vi "Add Parameter.vi"(8 "error in":errorcluster, 9 "parameter encoding":T1={"start index"=0, "size"=8, "encoding"=enum."BCD", "signed"=FALSE, "scale multiplier"=1.0, "scale offset"=0.0}, 10 "parameter definition":T4, 11 "label in":T3 format="%.0x") -> (0 "error out":errorcluster, 2 "parameter":T3 format="%.0x", 3 "label out":T3 format="%.0x")   [LabVIEW 2023, in "Ballard ARINC 429 Scripting.lvlib"]
doc: "Adds the specified <b>parameter definition</b> with <b>parameter encoding</b> to the system definition in the 'Word' subsection of <b>label in</b>. Returns the newly added <b>parameter</b> reference."
uses:
  Ballard ARINC 429 Scripting.lvlib
  <vilib>/NI VeriStand/Custom Device API/Custom Device Item Ref.ctl
  Shared/Parameter Definition.ctl
  <vilib>/NI/NI VeriStand Encoding and Decoding/Encoding.ctl
  <vilib>/NI VeriStand/Custom Device API/Custom Device Channel.ctl
  <vilib>/NI VeriStand/Custom Device API/Custom Device Channel Type.ctl
  Constants.vi
  <vilib>/NI VeriStand/Custom Device API/Custom Device API.lvlib
  ARINC 429/ARINC 429 Scripting.lvlib
  <vilib>/NI VeriStand/Custom Device Offline API/Custom Device Offline API.lvlib
  <vilib>/NI/NI VeriStand Encoding and Decoding/Encoding and Decoding.lvlib
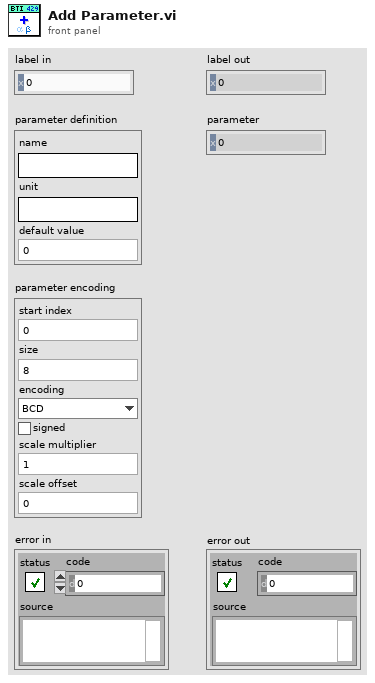
[diagram p1: front panel]
types:
  T1 = typedef "Parameter Definition.ctl" = cluster{"start index":i32, "size":i32, "encoding":T2, "signed":bool, "scale multiplier":dbl, "scale offset":dbl}
  T2 = typedef "Encoding and Decoding.lvlib/Encoding.ctl" = enum16{"BNR", "BCD", "Discrete"}
  T3 = typedef "Custom Device API.lvlib/Custom Device Item Ref.ctl" = u64
  T4 = cluster{"name":string, "unit":string, "default value":dbl}
  T5 = typedef "Custom Device API.lvlib/Custom Device Channel.ctl" = cluster{"Type":T6, "Units":string, "Default Value":dbl, "Faultable":bool, "Scalable":bool}
  T6 = typedef "Custom Device API.lvlib/Custom Device Channel Type.ctl" = enum16{"Input", "Output"}
  T7 = typedef "Direction.ctl" = enum16{"Rx", "Tx"}
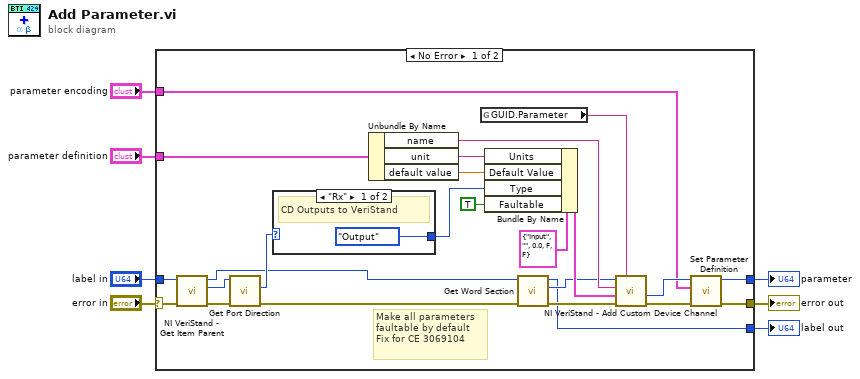
[diagram p0: block diagram]
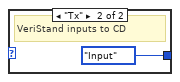
[diagram p2: hidden frame]
diagram:
  n1 = case shown="No Error" "error in" {
    selector: "error in" -> [w20 w35]
    tunnel: [w22 w35] -> w6
    tunnel: "label in" -> [w19 w34]
    tunnel: [w23 _] -> w4
    tunnel: "parameter definition" -> [w27 _]
    tunnel: [w9 w34] -> w2
    tunnel: "parameter encoding" -> [w11 _]
    frame No Error {
      # "Make all parameters faultable by default\nFix for CE 3069104"
      n2 = call <vilib>:"NI VeriStand - Get Item Parent.vi"("error in (no error)"=w20, "Item Ref in"=w19) -> ("error out"=w18:errorcluster, "Parent Ref"=w13:T3, "Item Ref out"=w12:T3)  [unwired: 6 in, 1 out]
      n3 = call "Get Port Direction.vi"("error in"=w18, "port ref in"=w13) -> ("error out"=w17:errorcluster, "direction"=w16:T7)  [unwired: 7 in, 1 out]
      n4 = case shown="\"Rx\"" w16 {
        tunnel: [Custom_Device_Channel_Type."Output" ("Type") Custom_Device_Channel_Type."Input" ("Type")] -> w15
        frame "Rx" {
          # "CD Outputs to VeriStand"
        }
        frame "Tx" {
          # "VeriStand inputs to CD"
        }
      }
      n5 = Unbundle By Name(w27) -> ("name"=w14:string, "unit"=w28:string, "default value"=w26:dbl)
      n6 = global read "Constants.vi" "GUID.Parameter"() -> (w31:string)
      n7 = Bundle By Name(cluster=T5 {"Type"=enum."Input", "Units"="", "Default Value"=0.0, "Faultable"=FALSE, "Scalable"=FALSE} ("Channel"), "Units"=w28, "Default Value"=w26, "Type"=w15, "Faultable"=TRUE) -> (w29:T5)
      n8 = call "Get Word Section.vi"("error in"=w17, "label ref"=w12) -> ("error out"=w21:errorcluster, "word ref"=w10:T3, "label ref out"=w9:T3)  [unwired: 7 in]
      n9 = call <vilib>:"NI VeriStand - Add Custom Device Channel.vi"("GUID (Default Channel)"=w31, "error in (no error)"=w21, "Channel"=w29, "Channel Name"=w14, "Parent Ref in"=w10) -> ("error out"=w25:errorcluster, "Channel Ref"=w24:T3)  [unwired: 3 in, 2 out]
      n10 = call "Set Parameter Definition.vi"("error in"=w25, "parameter definition"=w11, "parameter ref in"=w24) -> ("error out"=w22:errorcluster, "parameter ref out"=w23:T3)  [unwired: 7 in]
    }
    frame Error {
    }
  }
  "parameter" <- w4
  "error out" <- w6
  "label out" <- w2
